vi "Wire Encode Tag.vi"(7 "Field Number":i32, 10 "Wire Type":T1, 11 "Buffer in":u8[](array[numeric]) format="%.0x") -> (3 "Buffer":u8[](array[numeric]) format="%.0x")   [LabVIEW 2020, in "LV-Proto.lvlib"]
uses:
  LV-Proto.lvlib
  Wire Type.ctl
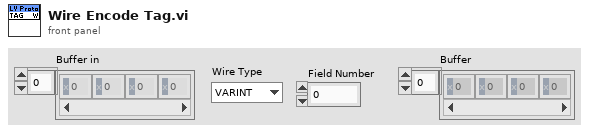
[diagram p1: front panel]
types:
  T1 = typedef "LV-Proto.lvlib/Wire Type.ctl" = enum8{"VARINT", "I64", "LEN", "SGROUP (Deprecated)", "EGROUP (Deprecated)", "I32"}
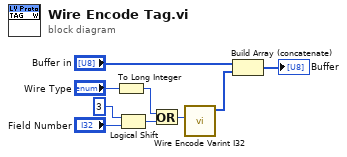
[diagram p0: block diagram]
diagram:
  n1 = To Long Integer(number="Wire Type") -> (32bit integer=w3:i32)
  n2 = Logical Shift(y=i16 3, x="Field Number") -> (x << y=w4:i32)
  n3 = Or(x=w3, y=w4) -> (x .or. y?=w2:i32)
  n4 = call "Wire Encode Varint I32.vi"("I32"=w2) -> ("Buffer"=w1:u8[])  [unwired: 10 in]
  n5 = Build Array (concatenate)("Buffer in", w1) -> (→"Buffer":u8[])
